vi "TrajectoryUtil_fromPathWeaverJSON.vi"(8 "error in (no error)":errorcluster, 11 "FileName":string="trajectory.json") -> (0 "error out":errorcluster, 3 "outTRAJECTORY":T2 {"States"."POSE"."ROTATION"."SIN" format="%13.4f"; "States"."POSE"."ROTATION"."COS" format="%13.4f"; "States"."POSE"."ROTATION"."VALUE" format="%13.4f"; "States"."POSE"."TRANSLATION"."Y" format="%14.3f"; "States"."POSE"."TRANSLATION"."X" format="%14.3f"; "TotalTImeSecs" format="%20.3f"}, 4 "Full Filename":string)   [LabVIEW 2019, in "Trajectory_Library.lvlib"]
doc: "Imports a Trajectory from a PathWeaver-style JSON file.\n\nParameters:\n - FileName - File name string of the json file to import from\n - Error In - Error cluster (not used)\n\nReturns:\n - Trajectory - Trajectory data structure\n - Error out - Returned error cluster"
uses:
  Trajectory_Library.lvlib
  TypeDef/TRAJECTORY.ctl
  TypeDef/TRAJ_STATE.ctl
  TypeDef/POSE2D.ctl
  TypeDef/TRANSLATION2D.ctl
  TypeDef/ROTATION2D.ctl
  Rotation2d_CreateAngle.vi
  Translation2d_Create.vi
panel:
  out "output":T1(array[cluster])
  in  "PathweaverJSON":T1(array[cluster])
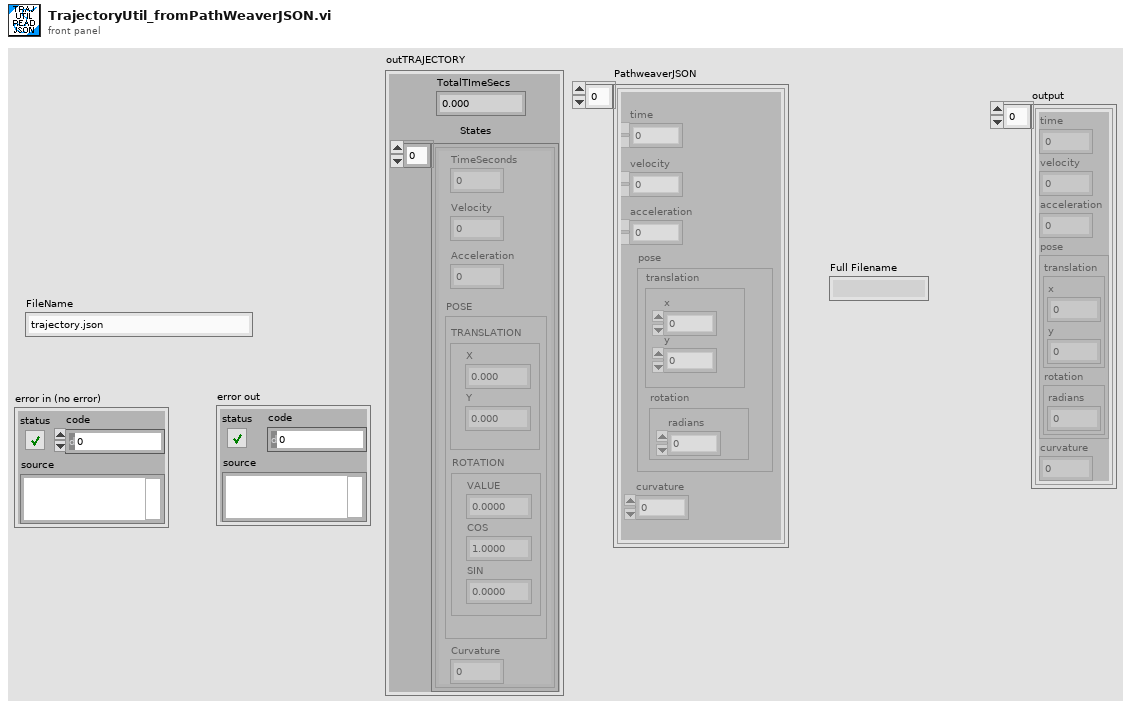
[diagram p1: front panel]
types:
  T1 = cluster{"time":dbl, "velocity":dbl, "acceleration":dbl, "pose":cluster{"translation":cluster{"x":dbl, "y":dbl}, "rotation":cluster{"radians":dbl}}, "curvature":dbl}[]
  T2 = typedef "Trajectory_Library.lvlib/TRAJECTORY.ctl" = cluster{"TotalTImeSecs":dbl, "States":T3[]}
  T3 = typedef "Trajectory_Library.lvlib/TRAJ_STATE.ctl" = cluster{"TimeSeconds":dbl, "Velocity":dbl, "Acceleration":dbl, "POSE":T4, "Curvature":dbl}
  T4 = typedef "Trajectory_Library.lvlib/POSE2D.ctl" = cluster{"TRANSLATION":T5, "ROTATION":T6}
  T5 = typedef "Trajectory_Library.lvlib/TRANSLATION2D.ctl" = cluster{"X":dbl, "Y":dbl}
  T6 = typedef "Trajectory_Library.lvlib/ROTATION2D.ctl" = cluster{"VALUE":dbl, "COS":dbl, "SIN":dbl}
  T7 = enum16{"open", "replace", "create", "open or create", "replace or create", "replace or create with confirmation"}
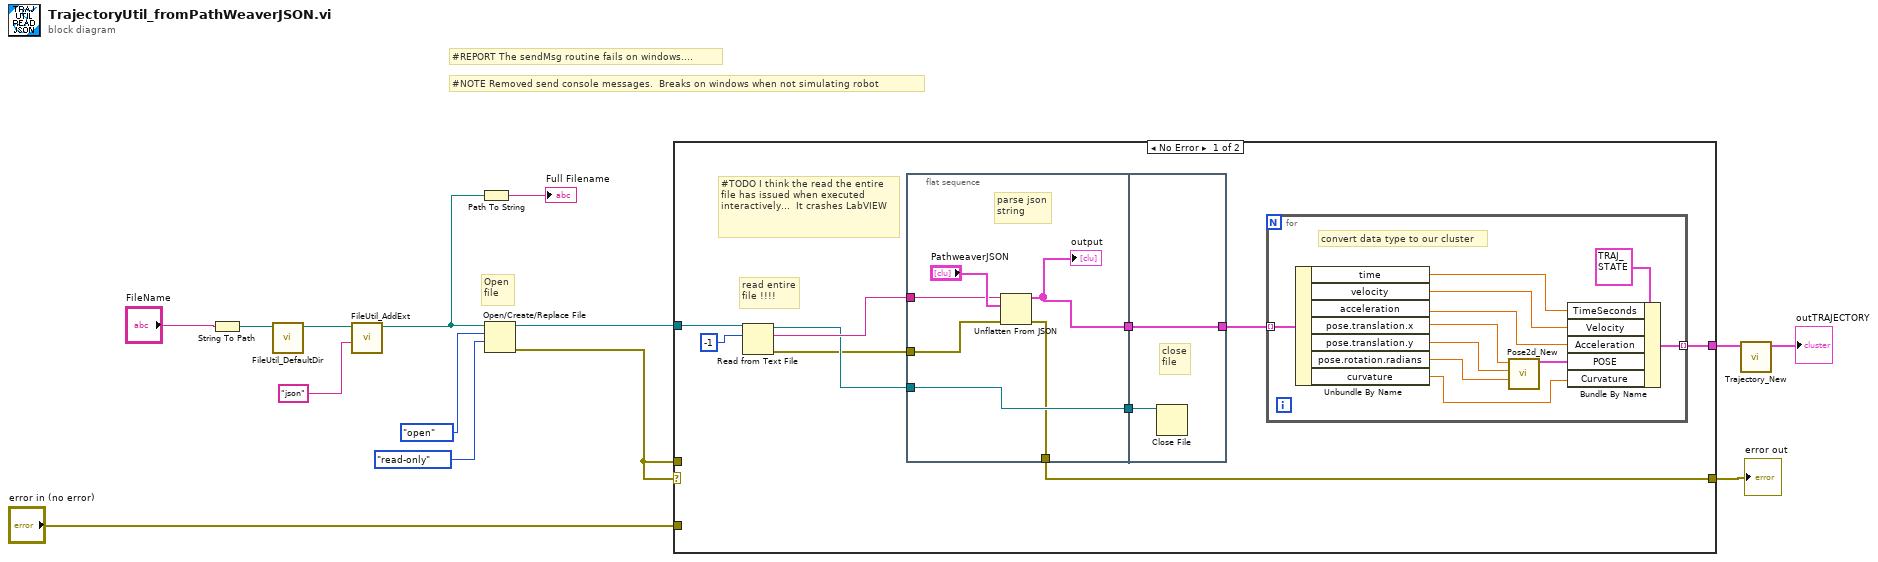
[diagram p0: block diagram]
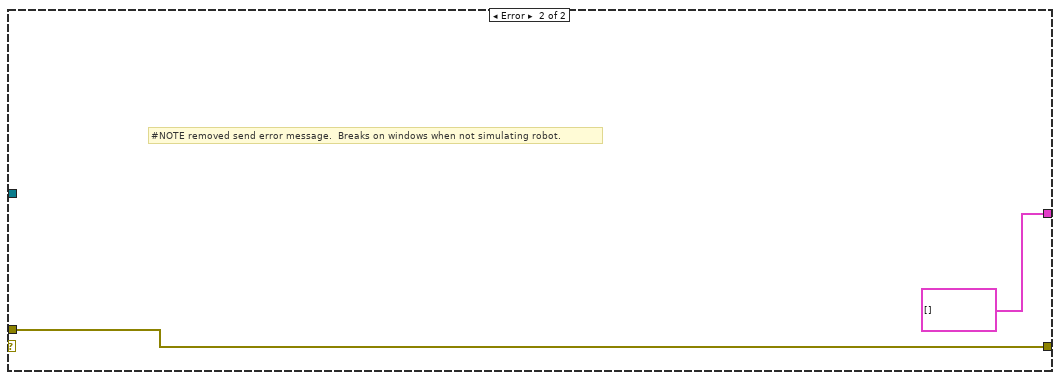
[diagram p2: hidden frame]
diagram:
  # "#NOTE Removed send console messages.  Breaks on windows when not simulating robot"
  # "#REPORT The sendMsg routine fails on windows...."
  # "Open\nfile"
  n1 = String To Path(string="FileName") -> (path=w4:path)
  n2 = call "FileUtil_DefaultDir.vi"("Path in"=w4) -> ("Path Out"=w3:path)  [unwired: 10 in]
  n3 = call "FileUtil_AddExt.vi"("Extension"="json", "Path in"=w3) -> ("Path out"=w1:path)  [unwired: 9 in]
  n4 = Path To String(path=w1) -> (string=→"Full Filename":string)
  n5 = Open/Create/Replace File(file path (use dialog)=w1, operation (0:open)=T7."open", access (0:read/write)=enum16{"read/write", "read-only", "write-only"}."read-only") -> (refnum out=w6:refnum<file>, error out=w12:errorcluster)  [unwired: 3 in, 1 out]
  n6 = case shown="No Error" w12 {
    tunnel: w6 -> [w23 _]
    tunnel: [w17 T3[] []] -> w11
    tunnel: w12 -> [_ w44]
    tunnel: [w16 w44] -> w8
    tunnel: "error in (no error)" -> [_ _]
    frame No Error {
      # "#TODO I think the read the entire\nfile has issued when executed\ninteractively...  It crashes LabVIEW"
      # "read entire\nfile !!!!"
      n7 = Read from Text File(file (use dialog)=w23, count=-1) -> (refnum out=w19:refnum<file>, text=w22:string, error out=w15:errorcluster)  [unwired: 2 in, 1 out]
      n8 = flat-sequence {
        tunnel: w22 -> [w29]
        tunnel: [w28] -> w20
        tunnel: w19 -> [w27]
        tunnel: [w27] -> w18
        tunnel: [w26] -> w16
        tunnel: w15 -> [w25]
        tunnel: [w32] -> w21
        tunnel: w20 -> [w32]
        tunnel: w18 -> [w31]
        frame #0 {
          # "parse json\nstring"
          n9 = Unflatten From JSON(JSON string=w29, type and defaults="PathweaverJSON", error in (no error)=w25) -> (value=w28:T1, error out=w26:errorcluster)  [unwired: 4 in]
          "output" <- w28
        }
        frame #1 {
          # "close\nfile"
          n10 = Close File(refnum=w31) -> ()  [unwired: 1 in, 2 out]
        }
      }
      n11 = for {
        tunnel: w21 -> [w43] mode=indexing
        tunnel: [w33] -> w17 mode=indexing
        # "convert data type to our cluster"
        n12 = Unbundle By Name(w43) -> ("time"=w40:dbl, "velocity"=w39:dbl, "acceleration"=w38:dbl, "pose.translation.x"=w37:dbl, "pose.translation.y"=w36:dbl, "pose.rotation.radians"=w35:dbl, "curvature"=w34:dbl)
        n13 = call "Pose2d_New.vi"("Heading"=w35, "Y"=w36, "X"=w37) -> ("out POSe"=w42:T4)  [unwired: 8 in]
        n14 = Bundle By Name(cluster=T3 {"TimeSeconds"=0.0, "Velocity"=0.0, "Acceleration"=0.0, "POSE"={"TRANSLATION"={"X"=0.0, "Y"=0.0}, "ROTATION"={"VALUE"=0.0, "COS"=1.0, "SIN"=0.0}}, "Curvature"=0.0} ("TRAJ_STATE"), "TimeSeconds"=w40, "Velocity"=w39, "Acceleration"=w38, "POSE"=w42, "Curvature"=w34) -> (w33:T3)
      }
    }
    frame Error {
      # "#NOTE removed send error message.  Breaks on windows when not simulating robot."
    }
  }
  "error out" <- w8
  n15 = call "Trajectory_New.vi"("TRAJ_STATES"=w11) -> ("TRAJECTORY"=→"outTRAJECTORY":T2)  [unwired: 10 in]
